vi "Module Init.vi"(8 "error in (no error)":errorcluster, 11 "SoftVar Module in":refnum<class "SoftVar Module.lvclass">) -> (0 "error out":errorcluster, 3 "SoftVar Module out":refnum<class "SoftVar Module.lvclass">)   [LabVIEW 2020, in "Volatus.lvlib" / "SoftVar Module.lvclass"]
uses:
  SoftVar Module.lvclass
  SoftVar Module.lvclass/SoftVar Module.ctl
  Module/Module.lvclass
  Message Registration.ctl
  Volatus.lvlib
  C:/dev/lv20CE/relink/lv-volatus/Volatus/Module/Module.lvclass
  C:/dev/lv20CE/relink/lv-volatus/Volatus/SoftVar Module/SoftVar Module.lvclass
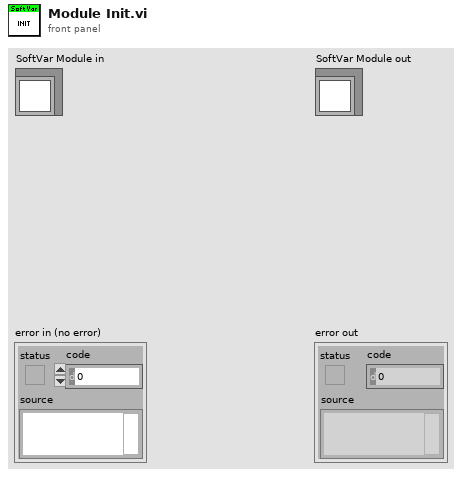
[diagram p1: front panel]
types:
  T1 = typedef "Volatus.lvlib/Message Registration.ctl" = cluster{"Message Type":string, "Message ID":string}
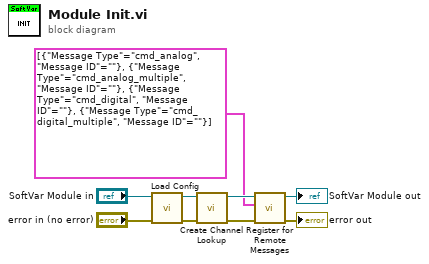
[diagram p0: block diagram]
diagram:
  n1 = call "Load Config.vi"("error in (no error)"="error in (no error)", "SoftVar Module in"="SoftVar Module in") -> ("error out"=w8:errorcluster, "SoftVar Module out"=w5:refnum<class "SoftVar Module.lvclass">)  [unwired: 8 in]
  n2 = call "Create Channel Lookup.vi"("error in (no error)"=w8, "SoftVar Module in"=w5) -> ("error out"=w6:errorcluster, "SoftVar Module out"=w3:refnum<class "SoftVar Module.lvclass">)  [unwired: 8 in]
  n3 = call "Register for Remote Messages.vi"("error in (no error)"=w6, "Messages"=T1[] [{"Message Type"="cmd_analog", "Message ID"=""}, {"Message Type"="cmd_analog_multiple", "Message ID"=""}, {"Message Type"="cmd_digital", "Message ID"=""}, {"Message Type"="cmd_digital_multiple", "Message ID"=""}], "Module in"=w3) -> ("error out"=→"error out":errorcluster, "Module out"=→"SoftVar Module out":refnum<class "SoftVar Module.lvclass">)  [unwired: 7 in]
